vi "Module Loop.vi"(8 "error in (no error)":errorcluster, 11 "Historian Charting Manager in":refnum<class "Historian Charting Manager.lvclass">) -> (0 "error out":errorcluster, 3 "Historian Charting Manager out":refnum<class "Historian Charting Manager.lvclass">)   [LabVIEW 2020, in "VolatusGUI.lvlib" / "Historian Charting Manager.lvclass"]
uses:
  Historian Charting Manager.lvclass
  C:/dev/lv20CE/relink/lv-volatus/Volatus/Module/Module.lvclass
  Volatus/Module/Module.lvclass/Module.ctl
  Volatus/MessageQ/MessageQ.lvclass/MessageQ.ctl
  Charting Config Value/Charting Config Value.lvclass
  Duplicate Group.ctl
  Volatus/Module/Module.lvclass
  Historian Charting Manager.lvclass/Historian Charting Manager.ctl
  JSON Charting Config.ctl
  JSON Chart Group.ctl
  JSON Plot Group.ctl
  JSON Plot Config.ctl
  New Plot Group Data.ctl
  VolatusConfig/VolatusConfigElement/VolatusConfigElement.lvclass
  Chart Info.ctl
  Volatus/MessageQ/MessageQ.lvclass
  Select Plot Group Data.ctl
  Plot Group Config.ctl
  X-Axis Type.ctl
  Plot Config.ctl
  Scale.ctl
  Chart Selection.ctl
  Chart Registration.ctl
  Plot Group Events Value/Plot Group Events Value.lvclass/Plot Group Events Value.ctl
  Plot Group Removed Data.ctl
  VolatusHistorian/Historian Identity/Historian Identity.lvclass
  C:/dev/lv20CE/relink/lv-volatus/Volatus/Identity/Identity.lvclass
  PluginGUI/PluginGUI.lvclass
  Chart GUI.vi
  <vilib>/Utility/error.llb/Error Cluster From Error Code.vi
  lv-promises/Promises/Promise/Promise.lvclass
  Plot Group Events Value/Plot Group Events Value.lvclass
  GUI Helper/GUI Helper.lvclass
  Volatus/Volatus.lvlib
  Volatus/VolatusAPI/VolatusAPI.lvclass
  C:/dev/lv20CE/relink/lv-volatus/VolatusGUI/Historian Charting Manager/Historian Charting Manager.lvclass
  VolatusGUI.lvlib
  GUI Info.ctl
  C:/dev/lv20CE/relink/lv-volatus/VolatusHistorian/Historian Identity/Historian Identity.lvclass
  C:/dev/lv20CE/relink/lv-volatus/VolatusGUI/PluginGUI/PluginGUI.lvclass
panel:
  out "Cover":string
  in  "Export":bool
  in  "Import":bool
  in  "New Chart":bool
  in  "Remove Group":bool
  in  "Dup Group":bool
  in  "New Group":bool
  in  "Chart Group":string(combo)
  # "To configure channels to plot, create a chart and then use the Config button in the upper right of the new chart window to create a plot group."
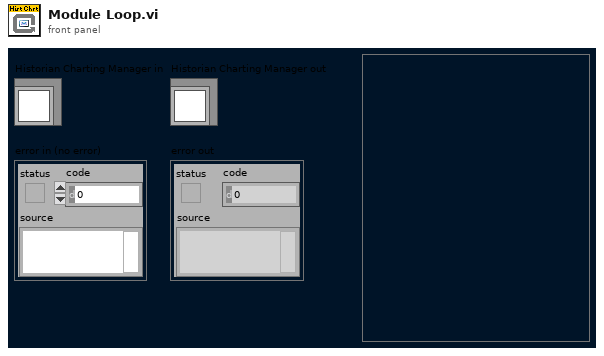
[diagram p1: front panel]
types:
  T1 = typedef "VolatusGUI.lvlib/Historian Charting Manager.lvclass/Duplicate Group.ctl" = cluster{"From":string, "Name":string}
  T2 = typedef "VolatusGUI.lvlib/JSON Charting Config.ctl" = cluster{"ChartGroups":T3[], "PlotGroups":T4[]}
  T3 = typedef "VolatusGUI.lvlib/JSON Chart Group.ctl" = cluster{"Name":string, "PlotGroups":string[]}
  T4 = typedef "VolatusGUI.lvlib/JSON Plot Group.ctl" = cluster{"Name":string, "Chart":cluster{"X-Axis":string, "X-Channel":string, "Now":bool, "Time":string, "SwapAxes":bool}, "Plots":T5[]}
  T5 = typedef "VolatusGUI.lvlib/JSON Plot Config.ctl" = cluster{"Channel":string, "Visible":bool, "Color":string, "Scale":string}
  T6 = enum32{"Invalid", "Standard", "Closed", "Hidden", "Minimized", "Maximized"}
  T7 = typedef "VolatusGUI.lvlib/GUI Info.ctl" = cluster{"Color":u32, "Name":string}
  T8 = enum8{"Enabled", "Disabled", "Disabled and Grayed Out"}
  T9 = typedef "VolatusGUI.lvlib/Historian Charting Manager.lvclass/New Plot Group Data.ctl" = cluster{"Name":string, "Plot Groups":string[]}
  T10 = typedef "VolatusGUI.lvlib/Historian Charting Manager.lvclass/Chart Info.ctl" = cluster{"PluginGUI":refnum<class "MessageQ.lvclass">, "Select Plot Group":refnum<user-event>}
  T11 = typedef "VolatusGUI.lvlib/Historian Charting Manager.lvclass/Select Plot Group Data.ctl" = cluster{"Chart Num":i32, "Plots Config":T12, "Plot Groups":string[]}
  T12 = typedef "VolatusGUI.lvlib/Historian Charting Manager.lvclass/Plot Group Config.ctl" = cluster{"Name":string, "X-Axis Type":T13, "X-Axis Channel":string, "Plots":T14[], "Lock Now":bool, "Time":string, "Swap Axes":bool}
  T13 = typedef "VolatusGUI.lvlib/Historian Charting Manager.lvclass/X-Axis Type.ctl" = enum16{"Time", "Channel"}
  T14 = typedef "VolatusGUI.lvlib/Historian Charting Manager.lvclass/Plot Config.ctl" = cluster{"Channel":string, "Visible":bool, "Color":u32, "Scale":T15}
  T15 = typedef "VolatusGUI.lvlib/Historian Charting Manager.lvclass/Scale.ctl" = enum16{"Left", "Right"}
  T16 = typedef "VolatusGUI.lvlib/Historian Charting Manager.lvclass/Chart Selection.ctl" = cluster{"Chart Num":i32, "Plot Group":string}
  T17 = typedef "VolatusGUI.lvlib/Historian Charting Manager.lvclass/Chart Registration.ctl" = cluster{"Chart Num":i32, "Select Plot Group":refnum<user-event>}
  T18 = typedef "VolatusGUI.lvlib/Historian Charting Manager.lvclass/Plot Group Removed Data.ctl" = cluster{"Name":string, "Plot Groups":string[]}
  T19 = typedef "VolatusGUI.lvlib/Historian Charting Manager.lvclass/Plot Group Events.ctl" = cluster{"Changed":refnum<user-event>, "Removed":refnum<user-event>, "New":refnum<user-event>, "Select":refnum<user-event>}
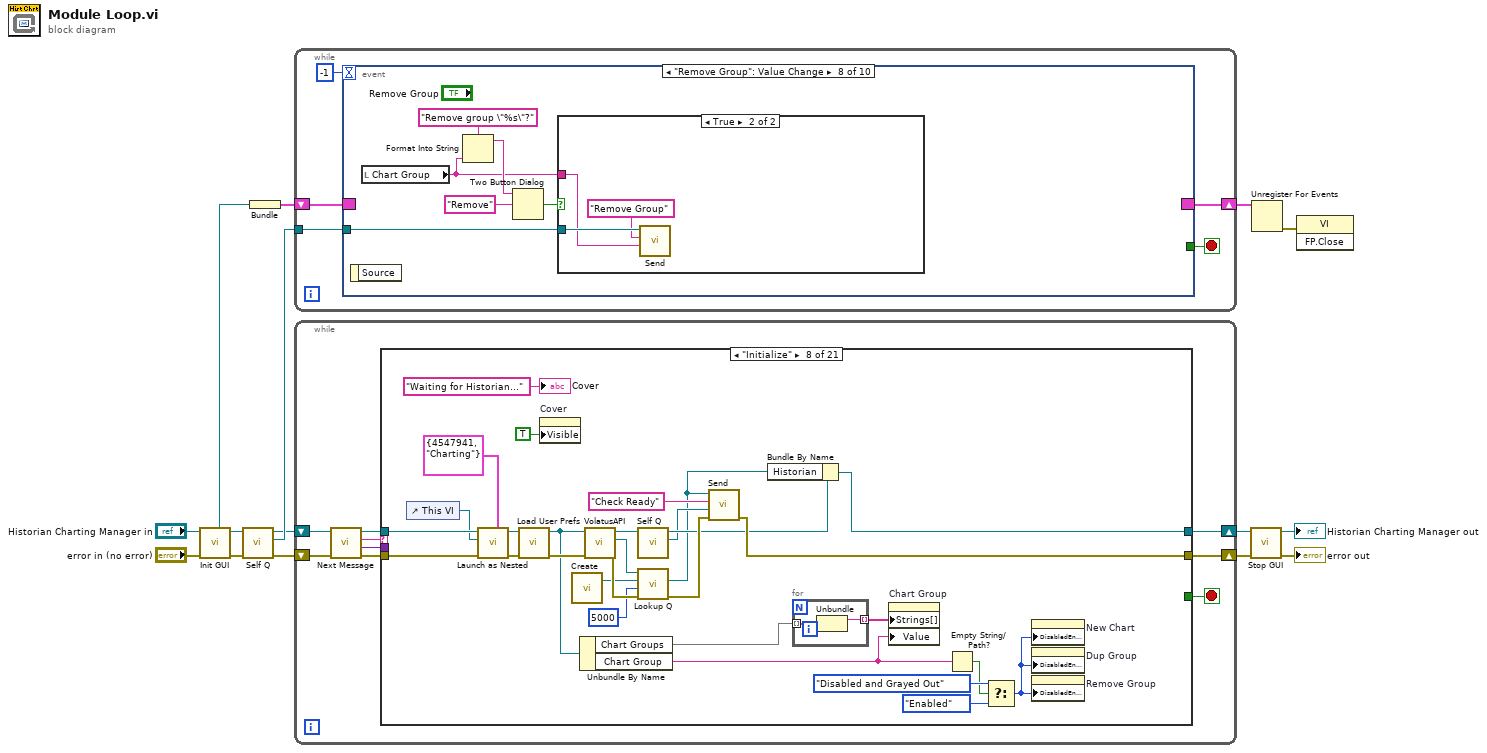
[diagram p0: block diagram]
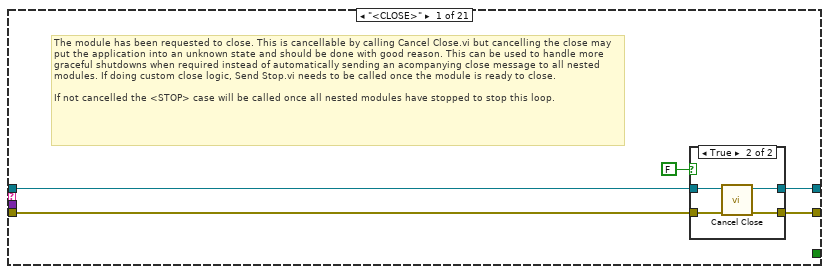
[diagram p2: hidden frame]
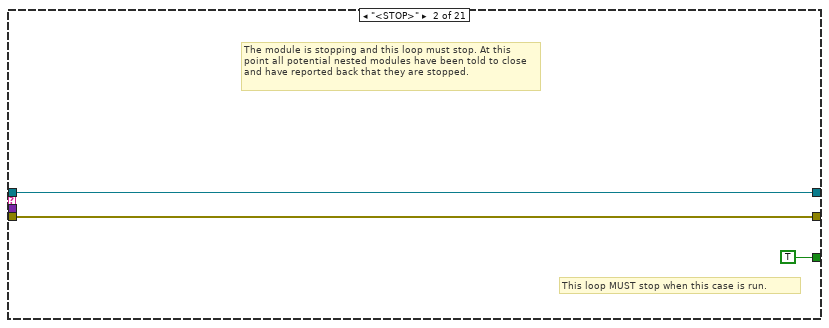
[diagram p4: hidden frame]
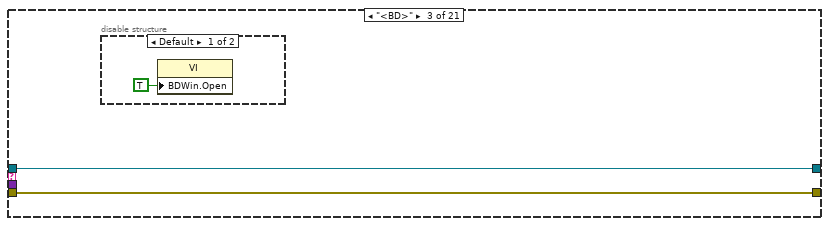
[diagram p5: hidden frame]
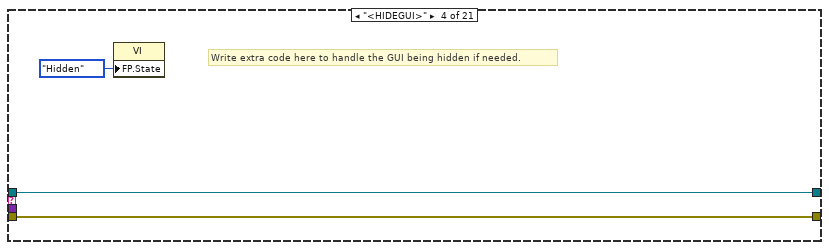
[diagram p7: hidden frame]
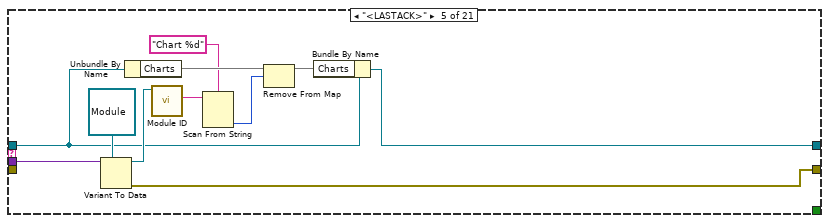
[diagram p8: hidden frame]
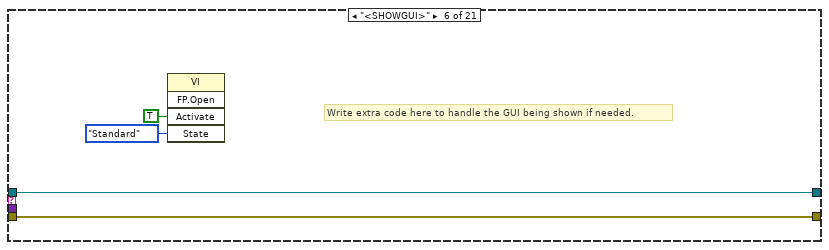
[diagram p9: hidden frame]
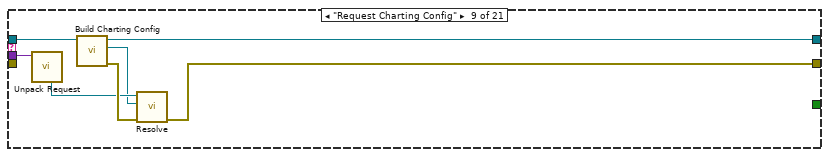
[diagram p11: hidden frame]
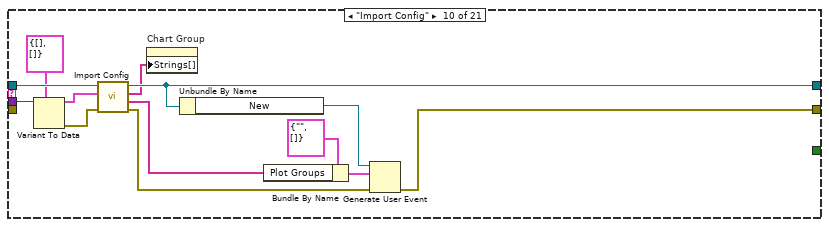
[diagram p12: hidden frame]
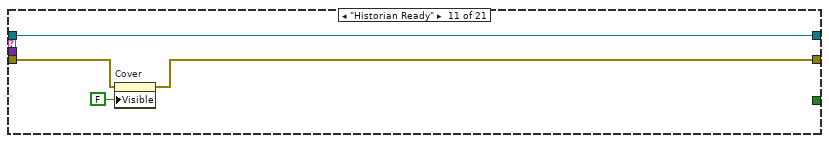
[diagram p13: hidden frame]
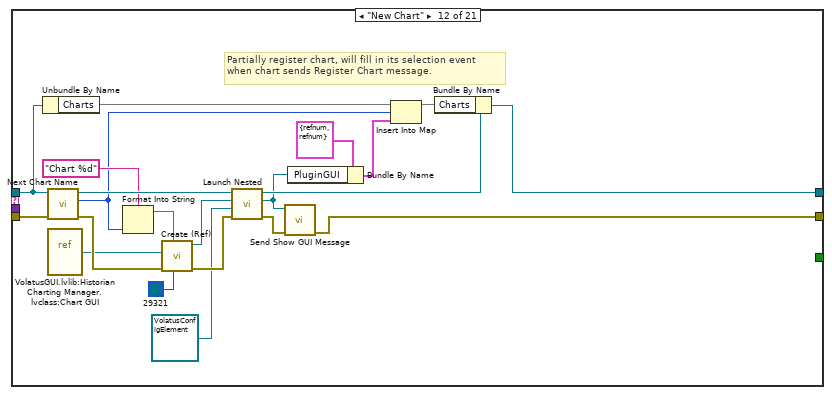
[diagram p14: hidden frame]
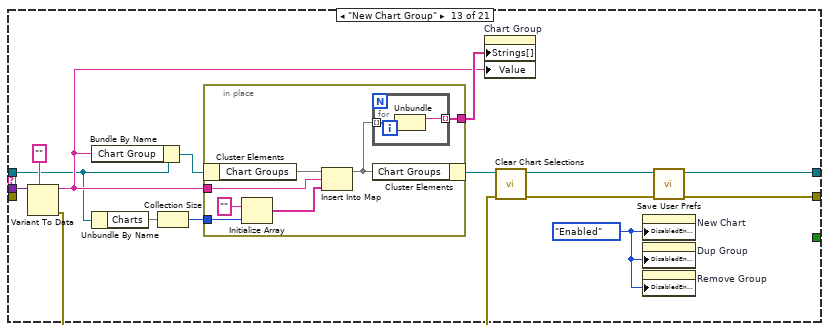
[diagram p15: hidden frame]
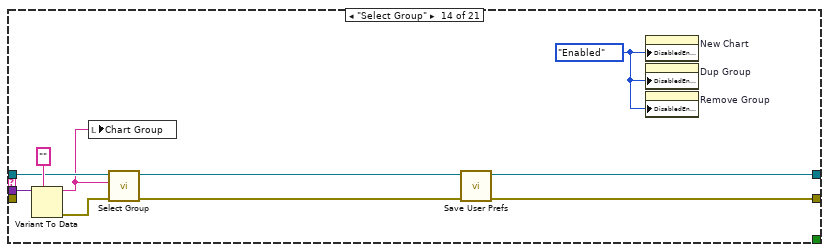
[diagram p16: hidden frame]
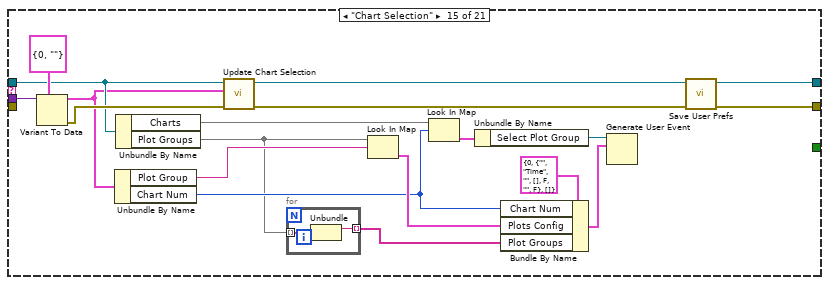
[diagram p17: hidden frame]
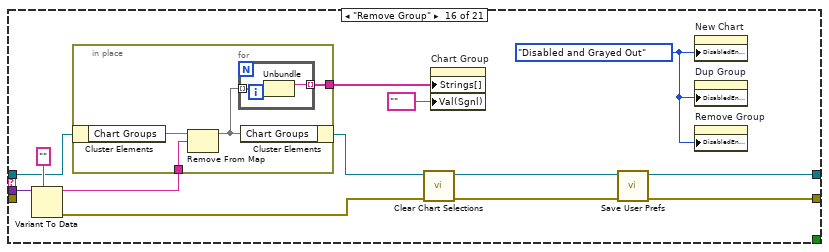
[diagram p18: hidden frame]
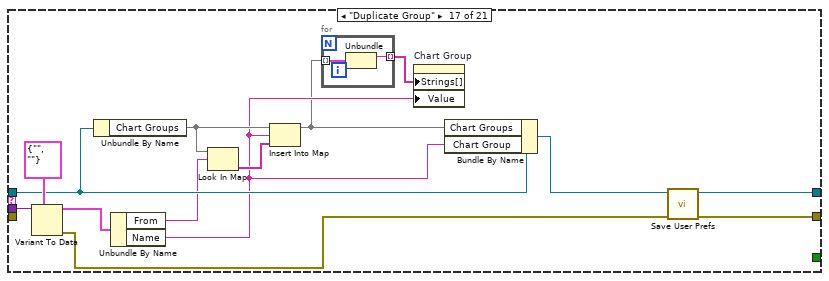
[diagram p19: hidden frame]
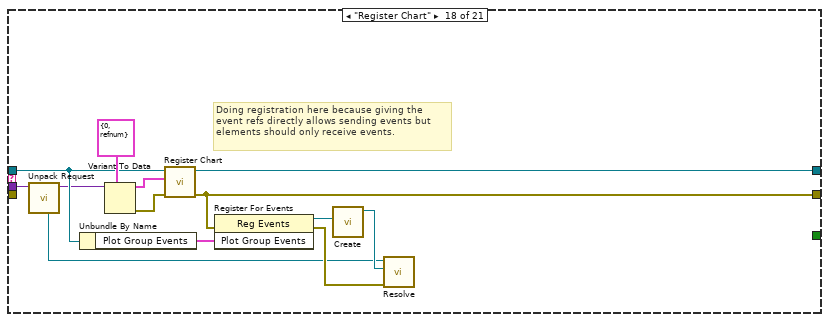
[diagram p20: hidden frame]
diagram:
  n1 = call "Init GUI.vi"("Module in"="Historian Charting Manager in") -> ("Module out"=w7:refnum<class "Historian Charting Manager.lvclass">, "Event Reg"=w12:refnum<event-registration>)  [unwired: 9 in]
  n2 = call "Self Q.vi"("Module in"=w7) -> ("Self Q"=w6:refnum<class "MessageQ.lvclass">, "Module out"=w5:refnum<class "Historian Charting Manager.lvclass">)  [unwired: 9 in]
  n3 = Bundle("Event Reg"=w12) -> (w8:cluster{"Event Reg":refnum<event-registration>})  [unwired: 1 in]
  n4 = while {
    tunnel: w6 -> [w18]
    shift-right: [w16] -> w9
    shift-left: w8 -> [w17]
    stop <- w15 stop-if-true
    n5 = event shown="[7] \"Remove Group\": Value Change" {
      selector: w17 -> [_ _ _ _ _ _ _ _ _ _]
      dyn-events: [_ _ _ _ _ _ _ _ _ _] -> w16
      timeout: -1 -> [_ _ _ _ _ _ _ _ _ _]
      tunnel: w18 -> [_ _ w22 w23 w30 w34 w44 w54 w63 w65]
      tunnel: [_ TRUE _ _ _ _ _ _ _ _] -> w15
      event Timeout {
        n6 = event-data() -> ()  [unwired: 1 in, 1 out]
      }
      event User Event {
        n7 = event-data() -> ()  [unwired: 1 in, 1 out]
      }
      event "Chart Group": Value Change {
        n8 = event-data() -> ("NewVal"=w21:string)  [unwired: 1 in]
        n9 = call "Send.vi"("Data"=w21, "ID"="Select Group", "MessageQ in"=w22) -> ()  [unwired: 7 in, 2 out]
      }
      event "Import": Value Change {
        # "Doing the prompt UI stuff here to allow other messages to still be handled by the QMH loop."
        n10 = event-data() -> ()  [unwired: 1 in, 1 out]
        n11 = call "Import Config UI.vi"() -> ("Config"=w24:T2, "Cancelled"=w25:bool)  [unwired: 10 in]
        n12 = case shown="False" w25 {
          tunnel: w24 -> [w27 _]
          tunnel: w23 -> [w28 _]
          frame False {
            n13 = call "Send.vi"("Data"=w27, "ID"="Import Config", "MessageQ in"=w28) -> ()  [unwired: 7 in, 2 out]
          }
          frame True {
          }
        }
      }
      event "Export": Value Change {
        n14 = event-data() -> ()  [unwired: 1 in, 1 out]
        n15 = call "Request.vi"("Response Type (None)"=refnum<class "Charting Config Value.lvclass"> refnum ("VolatusGUI:Charting Config Value.lvclass"), "ID"="Request Charting Config", "MessageQ in"=w30) -> ("Response"=w31:refnum<class "Charting Config Value.lvclass">)  [unwired: 6 in, 2 out]
        n16 = call "Read.vi"("Charting Config Value in"=w31) -> ("JSON Charting Config"=w29:T2)  [unwired: 10 in]
        n17 = call "Export Config UI.vi"("Config"=w29) -> ()  [unwired: 11 in]
      }
      event "New Group": Value Change {
        n18 = event-data() -> ()  [unwired: 1 in, 1 out]
        n19 = call "Group Name Prompt.vi"("Prompt"="Enter name for new group:") -> ("Cancelled"=w36:bool, "Name"=w35:string)  [unwired: 9 in]
        n20 = case shown="False" w36 {
          tunnel: w35 -> [w38 _]
          tunnel: w34 -> [w40 _]
          frame False {
            n21 = call "Send.vi"("Data"=w38, "ID"="New Chart Group", "MessageQ in"=w40) -> ()  [unwired: 7 in, 2 out]
          }
          frame True {
          }
        }
      }
      event "Dup Group": Value Change {
        n22 = event-data() -> ()  [unwired: 1 in, 1 out]
        n23 = local read "Chart Group"() -> (w42:string)
        n24 = Format Into String(format string="Enter new name for duplicated \"%s\" group:", w42) -> (resulting string=w41:string)  [unwired: 2 in, 1 out]
        n25 = call "Group Name Prompt.vi"("Prompt"=w41) -> ("Cancelled"=w45:bool, "Name"=w46:string)  [unwired: 9 in]
        n26 = case shown="False" w45 {
          tunnel: w46 -> [w50 _]
          tunnel: w44 -> [w49 _]
          tunnel: w42 -> [w51 _]
          frame False {
            n27 = Bundle By Name(cluster=T1 {"From"="", "Name"=""} ("Duplicate Group"), "From"=w51, "Name"=w50) -> (w48:T1)
            n28 = call "Send.vi"("Data"=w48, "ID"="Duplicate Group", "MessageQ in"=w49) -> ()  [unwired: 7 in, 2 out]
          }
          frame True {
          }
        }
      }
      event "Remove Group": Value Change {
        n29 = event-data() -> ()  [unwired: 1 in, 1 out]
        n30 = local read "Chart Group"() -> (w53:string)
        n31 = Format Into String(format string="Remove group \"%s\"?", w53) -> (resulting string=w56:string)  [unwired: 2 in, 1 out]
        n32 = Two Button Dialog(message=w56, 2:"Remove" ("T button name (\"OK\")")) -> (T button?=w55:bool)  [unwired: 1 in]
        n33 = case shown="True" w55 {
          tunnel: w54 -> [_ w61]
          tunnel: w53 -> [_ w59]
          frame False {
          }
          frame True {
            n34 = call "Send.vi"("Data"=w59, "ID"="Remove Group", "MessageQ in"=w61) -> ()  [unwired: 7 in, 2 out]
          }
        }
      }
      event "New Chart": Value Change {
        n35 = event-data() -> ()  [unwired: 1 in, 1 out]
        n36 = call "Send.vi"("ID"="New Chart", "MessageQ in"=w63) -> ()  [unwired: 8 in, 2 out]
      }
      event Panel Close? {
        n37 = event-data() -> ()  [unwired: 1 in, 1 out]
        n38 = call "Send.vi"("ID"="<HIDEGUI>", "MessageQ in"=w65) -> ()  [unwired: 8 in, 2 out]
        n39 = event-data("Discard?"=TRUE) -> ()  [unwired: 1 in, 1 out]
      }
    }
  }
  n40 = while {
    shift-right: [w70] -> w10
    shift-left: w5 -> [w75]
    shift-right: [w67] -> w11
    shift-left: "error in (no error)" -> [w74]
    stop <- w69 stop-if-true
    n41 = call "Next Message.vi"("error in (no error)"=w74, "Module in"=w75) -> ("error out"=w73:errorcluster, "Data"=w68:variant, "ID"=w72:string, "Module out"=w71:refnum<class "Historian Charting Manager.lvclass">)  [unwired: 6 in]
    n42 = case shown="\"Initialize\"" w72 {
      tunnel: w73 -> [w78 w88 w90 w94 _ w109 w111 w137 _ _ w164 w185 _ _ _ _ _ _ _ _ w321]
      tunnel: w71 -> [w79 w89 w91 w95 w101 w110 w112 w135 w147 w162 w166 w174 w190 w216 w225 w252 w273 w281 w299 w309 w319]
      tunnel: [w77 w89 w91 w95 w99 w110 w112 w117 w146 w157 w166 w171 w193 w212 w227 w244 w264 w286 w291 w301 w318] -> w70
      tunnel: [_ TRUE _ _ _ _ _ _ _ _ _ _ _ _ _ _ _ _ _ _ _] -> w69
      tunnel: w68 -> [_ _ _ _ w106 _ _ _ w148 w161 _ _ w202 w221 w239 w255 w275 w282 w298 w311 _]
      tunnel: [w76 w88 w90 w94 w104 w109 w111 w138 w143 w150 w163 w178 w195 w214 w226 w246 w262 w278 w293 w302 w320] -> w67
      frame "<CLOSE>" {
        # "The module has been requested to close. This is cancellable by calling Cancel Close.vi but cancelling the close may put the application into an unknown state and should be done with good reason. This can be used to handle more graceful shutdowns when required instead of automatically sending an acompanying close message to all nested modules. If doing custom close logic, Send Stop.vi needs to be called once the module is ready to close.\n\nIf not cancelled the <STOP> case will be called once all nested modules have stopped to stop this loop."
        n43 = case shown="True" FALSE {
          tunnel: w78 -> [w81 w86]
          tunnel: [w81 w85] -> w76
          tunnel: w79 -> [w82 w84]
          tunnel: [w82 w83] -> w77
          frame False {
          }
          frame True {
            n44 = call "Cancel Close.vi"("error in (no error)"=w86, "Module in"=w84) -> ("error out"=w85:errorcluster, "Module out"=w83:refnum<class "Historian Charting Manager.lvclass">)  [unwired: 8 in]
          }
        }
      }
      frame "<STOP>" {
        # "This loop MUST stop when this case is run."
        # "The module is stopping and this loop must stop. At this point all potential nested modules have been told to close and have reported back that they are stopped."
      }
      frame "<BD>" {
        n45 = disable-structure shown="Default" {
          frame condition #0 (active) {
            n46 = property class="VI"("BDWin.Open"=TRUE ("Block Diagram Window:Open")) -> ()  [unwired: 2 in, 2 out]
          }
          frame condition #1 {
          }
        }
      }
      frame "<HIDEGUI>" {
        # "Write extra code here to handle the GUI being hidden if needed."
        n47 = property class="VI"("FP.State"=T6."Hidden" ("Front Panel Window:State")) -> ()  [unwired: 2 in, 2 out]
      }
      frame "<LASTACK>" {
        n48 = Variant To Data(type=refnum<class "Module.lvclass"> refnum ("Volatus:Module"), Variant=w106) -> (data=w103:refnum<class "Module.lvclass">, error out=w104:errorcluster)  [unwired: 1 in]
        n49 = Unbundle By Name(w101) -> ("Charts"=w102:map{i32, T10})
        n50 = call-dynamic "Module ID.vi"("Module in"=w103) -> ("Module ID"=w98:string)  [unwired: 10 in]
        n51 = Scan From String(format string="Chart %d", input string=w98) -> (output 1=w96:i32)  [unwired: 3 in, 3 out]
        n52 = Remove From Map(10:w96, 11:w102) -> (3:w100:map{i32, T10})  [unwired: 2 out]
        n53 = Bundle By Name(cluster=w101, "Charts"=w100) -> (w99:refnum<class "Historian Charting Manager.lvclass">)
      }
      frame "<SHOWGUI>" {
        # "Write extra code here to handle the GUI being shown if needed."
        n54 = invoke class="VI" method="FP.Open"("Activate"=TRUE ("Activate?"), "State"=T6."Standard") -> ()  [unwired: 3 in, 5 out]
      }
      frame "<TIMEOUT>" {
        # "No message for this module was received in time"
      }
      frame "Initialize" {
        n55 = control-ref of="This VI"() -> (w134:refnum<vi>)
        n56 = call "Launch as Nested.vi"("GUI Info (Default)"=T7 {"Color"=4547941, "Name"="Charting"}, "error in (no error)"=w137, "GUI"=w134, "Parent in"=w135) -> ("error out"=w136:errorcluster, "Parent"=w133:refnum<class "Historian Charting Manager.lvclass">)  [unwired: 5 in, 1 out]
        n57 = call "Load User Prefs.vi"("error in (no error)"=w136, "Historian Charting Manager in"=w133) -> ("error out"=w139:errorcluster, "Historian Charting Manager out"=w126:refnum<class "Historian Charting Manager.lvclass">)  [unwired: 8 in]
        n58 = property on="Cover" class="Str"("Visible"=TRUE) -> ()  [unwired: 2 in, 2 out]
        n59 = call "Create.vi"() -> ("Historian Identity out"=w120:refnum<class "Historian Identity.lvclass">)  [unwired: 7 in]
        n60 = Unbundle By Name(w126) -> ("Chart Groups"=w132:map{string, string[]}, "Chart Group"=w128:string)
        n61 = call "VolatusAPI.vi"("Module in"=w126) -> ("VolatusAPI"=w118:refnum<class "VolatusAPI.lvclass">, "Module out"=w119:refnum<class "Historian Charting Manager.lvclass">)  [unwired: 9 in]
        n62 = call "Self Q.vi"("Module in"=w119) -> ("Self Q"=w124:refnum<class "MessageQ.lvclass">, "Module out"=w125:refnum<class "Historian Charting Manager.lvclass">)  [unwired: 9 in]
        n63 = call "Lookup Q.vi"("error in (no error)"=w139, "Timeout ms (0)"=5000, "Identity"=w120, "VolatusAPI in"=w118) -> ("error out"=w140:errorcluster, "MessageQ"=w116:refnum<class "MessageQ.lvclass">)  [unwired: 5 in, 1 out]
        n64 = call "Send.vi"("error in (no error)"=w140, "Data"=w124, "ID"="Check Ready", "MessageQ in"=w116) -> ("error out"=w138:errorcluster)  [unwired: 6 in, 1 out]
        n65 = Bundle By Name(cluster=w125, "Historian"=w116) -> (w117:refnum<class "Historian Charting Manager.lvclass">)
        n66 = for {
          tunnel: w132 -> [w142] mode=indexing
          tunnel: [w141] -> w131 mode=indexing
          n67 = Unbundle(w142) -> ("Chart Group"=w141:string)  [unwired: 1 out]
        }
        n68 = property on="Chart Group" class="CmbBox"("Strings[]"=w131, "Value"=w128) -> ()  [unwired: 2 in, 2 out]
        n69 = Empty String/Path?(string/path=w128) -> (empty?=w127:bool)
        n70 = Select(t=T8."Disabled and Grayed Out" ("Disabled"), s=w127, f=T8."Enabled") -> (s? t:f=w114:T8)
        n71 = property on="New Chart" class="Bool"("DisabledEnum"=w114) -> ()  [unwired: 2 in, 2 out]
        n72 = property on="Dup Group" class="Bool"("DisabledEnum"=w114) -> ()  [unwired: 2 in, 2 out]
        n73 = property on="Remove Group" class="Bool"("DisabledEnum"=w114) -> ()  [unwired: 2 in, 2 out]
        "Cover" <- "Waiting for Historian..." ("Cover")
      }
      frame "Request Charting Config" {
        n74 = call "Unpack Request.vi"("Request Data"=w148) -> ("Promise"=w145:refnum<class "Promise.lvclass">)  [unwired: 8 in, 2 out]
        n75 = call "Build Charting Config.vi"("Historian Charting Manager in"=w147) -> ("error out"=w149:errorcluster, "Charting Config Value"=w144:refnum<class "Charting Config Value.lvclass">, "Historian Charting Manager out"=w146:refnum<class "Historian Charting Manager.lvclass">)  [unwired: 8 in]
        n76 = call "Resolve.vi"("error in (no error)"=w149, "Result (None)"=w144, "Promise in"=w145) -> ("error out"=w143:errorcluster)  [unwired: 7 in, 1 out]
      }
      frame "Import Config" {
        n77 = Variant To Data(type=T2 {"ChartGroups"=[], "PlotGroups"=[]} ("JSON Charting Config"), Variant=w161) -> (data=w159:T2, error out=w158:errorcluster)  [unwired: 1 in]
        n78 = call "Import Config.vi"("error in (no error)"=w158, "JSON Charting Config"=w159, "Historian Charting Manager in"=w162) -> ("error out"=w151:errorcluster, "Plot Groups"=w153:string[], "Chart Groups"=w152:string[], "Historian Charting Manager out"=w157:refnum<class "Historian Charting Manager.lvclass">)  [unwired: 5 in]
        n79 = property on="Chart Group" class="CmbBox"("Strings[]"=w152) -> ()  [unwired: 2 in, 2 out]
        n80 = Unbundle By Name(w157) -> ("New"=w156:refnum<user-event>)
        n81 = Bundle By Name(cluster=T9 {"Name"="", "Plot Groups"=[]} ("event data"), "Plot Groups"=w153) -> (w154:T9)
        n82 = Generate User Event(user event=w156, event data cluster=w154, error in=w151) -> (error out=w150:errorcluster)  [unwired: 1 in, 1 out]
      }
      frame "Historian Ready" {
        n83 = property on="Cover" class="Str"(error in=w164, "Visible"=FALSE) -> (error out=w163:errorcluster)  [unwired: 1 in, 1 out]
      }
      frame "New Chart" {
        # "Partially register chart, will fill in its selection event when chart sends Register Chart message."
        n84 = Unbundle By Name(w174) -> ("Charts"=w173:map{i32, T10})
        n85 = call "Next Chart Name.vi"("error in (no error)"=w185, "Historian Charting Manager in"=w174) -> ("error out"=w186:errorcluster, "Next Chart Num"=w169:i32, "Historian Charting Manager out"=w183:refnum<class "Historian Charting Manager.lvclass">)  [unwired: 7 in]
        n86 = vi-ref "VolatusGUI.lvlib:Historian Charting Manager.lvclass:Chart GUI.vi"() -> (w184:refnum<vi>)
        n87 = Format Into String(format string="Chart %d", w169) -> (resulting string=w175:string)  [unwired: 2 in, 1 out]
        n88 = call "Create (Ref).vi"("Color (Default)"=u32 29321, "Name"=w175, "error in (no error)"=w186, "VI"=w184) -> ("error out"=w187:errorcluster, "PluginGUI out"=w182:refnum<class "PluginGUI.lvclass">)  [unwired: 6 in]
        n89 = call "Launch Nested.vi"("error in (no error)"=w187, "Config Element"=refnum<class "VolatusConfigElement.lvclass"> refnum, "Nested Module"=w182, "Parent in"=w183) -> ("error out"=w179:errorcluster, "MessageQ"=w167:refnum<class "MessageQ.lvclass">, "Parent out"=w180:refnum<class "Historian Charting Manager.lvclass">)  [unwired: 5 in]
        n90 = call "Send Show GUI Message.vi"("error in (no error)"=w179, "MessageQ"=w167) -> ("error out"=w178:errorcluster)  [unwired: 9 in]
        n91 = Bundle By Name(cluster=T10 {"PluginGUI"=refnum, "Select Plot Group"=refnum} ("value"), "PluginGUI"=w167) -> (w168:T10)
        n92 = Insert Into Map(map in=w173, key=w169, value=w168) -> (map out=w170:map{i32, T10})  [unwired: 2 out]
        n93 = Bundle By Name(cluster=w180, "Charts"=w170) -> (w171:refnum<class "Historian Charting Manager.lvclass">)
      }
      frame "New Chart Group" {
        w192 = T8."Enabled" ("Disabled")
        n94 = Variant To Data(type="", Variant=w202) -> (data=w191:string, error out=w200:errorcluster)  [unwired: 1 in]
        n95 = Bundle By Name(cluster=w190, "Chart Group"=w191) -> (w196:refnum<class "Historian Charting Manager.lvclass">)
        n96 = Unbundle By Name(w190) -> ("Charts"=w189:map{i32, T10})
        n97 = Collection Size(1:w189) -> (0:w188:i32)
        n98 = in-place {
          in-place-border: w191 -> [w208]
          in-place-border: [w206] -> w197
          in-place-border: w188 -> [w205]
          n99 = in-place-cluster #1(w196) -> ("Chart Groups"=w209:map{string, string[]})
          n100 = Initialize Array("", w205) -> (w203:string[])
          n101 = Insert Into Map(map in=w209, key=w208, value=w203) -> (map out=w207:map{string, string[]})  [unwired: 2 out]
          n102 = for {
            tunnel: w207 -> [w211] mode=indexing
            tunnel: [w210] -> w206 mode=indexing
            n103 = Unbundle(w211) -> ("Chart Group"=w210:string)  [unwired: 1 out]
          }
          n104 = in-place-cluster #1("Chart Groups"=w207) -> (w198:refnum<class "Historian Charting Manager.lvclass">)
        }
        n105 = property on="Chart Group" class="CmbBox"("Strings[]"=w197, "Value"=w191) -> ()  [unwired: 2 in, 2 out]
        n106 = call "Clear Chart Selections.vi"("error in (no error)"=w200, "Historian Charting Manager in"=w198) -> ("error out"=w199:errorcluster, "Historian Charting Manager out"=w194:refnum<class "Historian Charting Manager.lvclass">)  [unwired: 8 in]
        n107 = property on="New Chart" class="Bool"("DisabledEnum"=w192) -> ()  [unwired: 2 in, 2 out]
        n108 = property on="Dup Group" class="Bool"("DisabledEnum"=w192) -> ()  [unwired: 2 in, 2 out]
        n109 = property on="Remove Group" class="Bool"("DisabledEnum"=w192) -> ()  [unwired: 2 in, 2 out]
        n110 = call "Save User Prefs.vi"("error in (no error)"=w199, "Historian Charting Manager in"=w194) -> ("error out"=w195:errorcluster, "Historian Charting Manager out"=w193:refnum<class "Historian Charting Manager.lvclass">)  [unwired: 8 in]
      }
      frame "Select Group" {
        w219 = T8."Enabled" ("Disabled")
        n111 = Variant To Data(type="", Variant=w221) -> (data=w215:string, error out=w218:errorcluster)  [unwired: 1 in]
        n112 = local write "Chart Group"(w215) -> ()
        n113 = call "Select Group.vi"("error in (no error)"=w218, "Group (Empty = none)"=w215, "Historian Charting Manager in"=w216) -> ("error out"=w217:errorcluster, "Historian Charting Manager out"=w213:refnum<class "Historian Charting Manager.lvclass">)  [unwired: 7 in]
        n114 = call "Save User Prefs.vi"("error in (no error)"=w217, "Historian Charting Manager in"=w213) -> ("error out"=w214:errorcluster, "Historian Charting Manager out"=w212:refnum<class "Historian Charting Manager.lvclass">)  [unwired: 8 in]
        n115 = property on="New Chart" class="Bool"("DisabledEnum"=w219) -> ()  [unwired: 2 in, 2 out]
        n116 = property on="Dup Group" class="Bool"("DisabledEnum"=w219) -> ()  [unwired: 2 in, 2 out]
        n117 = property on="Remove Group" class="Bool"("DisabledEnum"=w219) -> ()  [unwired: 2 in, 2 out]
      }
      frame "Chart Selection" {
        n118 = Variant To Data(type=T16 {"Chart Num"=0, "Plot Group"=""} ("Chart Selection"), Variant=w239) -> (data=w222:T16, error out=w240:errorcluster)  [unwired: 1 in]
        n119 = Unbundle By Name(w222) -> ("Plot Group"=w231:string, "Chart Num"=w230:i32)
        n120 = Unbundle By Name(w225) -> ("Charts"=w237:map{i32, T10}, "Plot Groups"=w229:map{string, T12})
        n121 = call "Update Chart Selection.vi"("error in (no error)"=w240, "Chart Selection"=w222, "Historian Charting Manager in"=w225) -> ("error out"=w224:errorcluster, "Historian Charting Manager out"=w223:refnum<class "Historian Charting Manager.lvclass">)  [unwired: 7 in]
        n122 = for {
          tunnel: w229 -> [w242] mode=indexing
          tunnel: [w241] -> w228 mode=indexing
          n123 = Unbundle(w242) -> ("Name"=w241:string)  [unwired: 1 out]
        }
        n124 = Look In Map(map=w229, key=w231) -> (value=w232:T12)  [unwired: 1 in, 1 out]
        n125 = Look In Map(map=w237, key=w230) -> (value=w236:T10)  [unwired: 1 in, 1 out]
        n126 = Unbundle By Name(w236) -> ("Select Plot Group"=w235:refnum<user-event>)
        n127 = Bundle By Name(cluster=T11 {"Chart Num"=0, "Plots Config"={"Name"="", "X-Axis Type"=enum."Time", "X-Axis Channel"="", "Plots"=[], "Lock Now"=FALSE, "Time"="", "Swap Axes"=FALSE}, "Plot Groups"=[]} ("event data"), "Chart Num"=w230, "Plots Config"=w232, "Plot Groups"=w228) -> (w233:T11)
        n128 = Generate User Event(user event=w235, event data cluster=w233) -> ()  [unwired: 2 in, 2 out]
        n129 = call "Save User Prefs.vi"("error in (no error)"=w224, "Historian Charting Manager in"=w223) -> ("error out"=w226:errorcluster, "Historian Charting Manager out"=w227:refnum<class "Historian Charting Manager.lvclass">)  [unwired: 8 in]
      }
      frame "Remove Group" {
        w253 = T8."Disabled and Grayed Out" ("Disabled")
        n130 = Variant To Data(type="", Variant=w255) -> (data=w251:string, error out=w249:errorcluster)  [unwired: 1 in]
        n131 = in-place {
          in-place-border: w251 -> [w258]
          in-place-border: [w256] -> w243
          n132 = in-place-cluster #2(w252) -> ("Chart Groups"=w259:map{string, string[]})
          n133 = Remove From Map(10:w258, 11:w259) -> (3:w257:map{string, string[]})  [unwired: 2 out]
          n134 = for {
            tunnel: w257 -> [w261] mode=indexing
            tunnel: [w260] -> w256 mode=indexing
            n135 = Unbundle(w261) -> ("Chart Group"=w260:string)  [unwired: 1 out]
          }
          n136 = in-place-cluster #2("Chart Groups"=w257) -> (w250:refnum<class "Historian Charting Manager.lvclass">)
        }
        n137 = call "Clear Chart Selections.vi"("error in (no error)"=w249, "Historian Charting Manager in"=w250) -> ("error out"=w248:errorcluster, "Historian Charting Manager out"=w245:refnum<class "Historian Charting Manager.lvclass">)  [unwired: 8 in]
        n138 = property on="Chart Group" class="CmbBox"("Strings[]"=w243, "Val(Sgnl)"="" ("Chart Group")) -> ()  [unwired: 2 in, 2 out]
        n139 = call "Save User Prefs.vi"("error in (no error)"=w248, "Historian Charting Manager in"=w245) -> ("error out"=w246:errorcluster, "Historian Charting Manager out"=w244:refnum<class "Historian Charting Manager.lvclass">)  [unwired: 8 in]
        n140 = property on="New Chart" class="Bool"("DisabledEnum"=w253) -> ()  [unwired: 2 in, 2 out]
        n141 = property on="Dup Group" class="Bool"("DisabledEnum"=w253) -> ()  [unwired: 2 in, 2 out]
        n142 = property on="Remove Group" class="Bool"("DisabledEnum"=w253) -> ()  [unwired: 2 in, 2 out]
      }
      frame "Duplicate Group" {
        n143 = Variant To Data(type=T1 {"From"="", "Name"=""} ("Duplicate Group"), Variant=w275) -> (data=w272:T1, error out=w263:errorcluster)  [unwired: 1 in]
        n144 = Unbundle By Name(w273) -> ("Chart Groups"=w270:map{string, string[]})
        n145 = Unbundle By Name(w272) -> ("From"=w271:string, "Name"=w267:string)
        n146 = Look In Map(map=w270, key=w271) -> (value=w269:string[])  [unwired: 1 in, 1 out]
        n147 = Insert Into Map(map in=w270, key=w267, value=w269) -> (map out=w266:map{string, string[]})  [unwired: 2 out]
        n148 = for {
          tunnel: w266 -> [w277] mode=indexing
          tunnel: [w276] -> w265 mode=indexing
          n149 = Unbundle(w277) -> ("Chart Group"=w276:string)  [unwired: 1 out]
        }
        n150 = property on="Chart Group" class="CmbBox"("Strings[]"=w265, "Value"=w267) -> ()  [unwired: 2 in, 2 out]
        n151 = Bundle By Name(cluster=w273, "Chart Groups"=w266, "Chart Group"=w267) -> (w268:refnum<class "Historian Charting Manager.lvclass">)
        n152 = call "Save User Prefs.vi"("error in (no error)"=w263, "Historian Charting Manager in"=w268) -> ("error out"=w262:errorcluster, "Historian Charting Manager out"=w264:refnum<class "Historian Charting Manager.lvclass">)  [unwired: 8 in]
      }
      frame "Register Chart" {
        # "Doing registration here because giving the event refs directly allows sending events but elements should only receive events."
        n153 = call "Unpack Request.vi"("Request Data"=w282) -> ("Data"=w280:variant, "Promise"=w279:refnum<class "Promise.lvclass">)  [unwired: 8 in, 1 out]
        n154 = Unbundle By Name(w281) -> ("Plot Group Events"=w284:T19)
        n155 = Variant To Data(type=T17 {"Chart Num"=0, "Select Plot Group"=refnum} ("Chart Registration"), Variant=w280) -> (data=w288:T17, error out=w287:errorcluster)  [unwired: 1 in]
        n156 = call "Register Chart.vi"("error in (no error)"=w287, "Chart Registration"=w288, "Historian Charting Manager in"=w281) -> ("error out"=w278:errorcluster, "Historian Charting Manager out"=w286:refnum<class "Historian Charting Manager.lvclass">)  [unwired: 7 in]
        n157 = register-events(error in=w278, w284) -> (reference out=w283:refnum<event-registration>, error out=w290:errorcluster)  [unwired: 1 in]
        n158 = call "Create.vi"("Plot Group"=w283) -> ("Plot Group Events Value out"=w285:refnum<class "Plot Group Events Value.lvclass">)  [unwired: 10 in]
        n159 = call "Resolve.vi"("error in (no error)"=w290, "Result (None)"=w285, "Promise in"=w279) -> ()  [unwired: 7 in, 2 out]
      }
      frame "Update Plots Config" {
        n160 = Variant To Data(type=T12 {"Name"="", "X-Axis Type"=enum."Time", "X-Axis Channel"="", "Plots"=[], "Lock Now"=FALSE, "Time"="", "Swap Axes"=FALSE} ("Plot Group Config"), Variant=w298) -> (data=w296:T12, error out=w295:errorcluster)  [unwired: 1 in]
        n161 = call "Update Plots Config.vi"("error in (no error)"=w295, "Plot Group Config"=w296, "Historian Charting Manager in"=w299) -> ("error out"=w294:errorcluster, "Historian Charting Manager out"=w292:refnum<class "Historian Charting Manager.lvclass">)  [unwired: 7 in]
        n162 = call "Save User Prefs.vi"("error in (no error)"=w294, "Historian Charting Manager in"=w292) -> ("error out"=w293:errorcluster, "Historian Charting Manager out"=w291:refnum<class "Historian Charting Manager.lvclass">)  [unwired: 8 in]
      }
      frame "Remove Plot Group" {
        n163 = Variant To Data(type="", Variant=w311) -> (data=w303:string)  [unwired: 1 in, 1 out]
        n164 = in-place {
          in-place-border: w303 -> [w314]
          in-place-border: [w312] -> w304
          n165 = in-place-cluster #3(w309) -> ("Plot Groups"=w315:map{string, T12})
          n166 = Remove From Map(10:w314, 11:w315) -> (3:w313:map{string, T12})  [unwired: 2 out]
          n167 = in-place-cluster #3("Plot Groups"=w313) -> (w300:refnum<class "Historian Charting Manager.lvclass">)
          n168 = for {
            tunnel: w313 -> [w317] mode=indexing
            tunnel: [w316] -> w312 mode=indexing
            n169 = Unbundle(w317) -> ("Name"=w316:string)  [unwired: 1 out]
          }
        }
        n170 = Bundle By Name(cluster=T18 {"Name"="", "Plot Groups"=[]} ("event data"), "Plot Groups"=w304, "Name"=w303) -> (w306:T18)
        n171 = Unbundle By Name(w300) -> ("Removed"=w308:refnum<user-event>)
        n172 = Generate User Event(user event=w308, event data cluster=w306) -> (error out=w305:errorcluster)  [unwired: 2 in, 1 out]
        n173 = call "Save User Prefs.vi"("error in (no error)"=w305, "Historian Charting Manager in"=w300) -> ("error out"=w302:errorcluster, "Historian Charting Manager out"=w301:refnum<class "Historian Charting Manager.lvclass">)  [unwired: 8 in]
      }
      frame Default {
        n174 = call "Report Unhandled Message ID.vi"("error in (no error)"=w321, "Module in"=w319) -> ("error out"=w320:errorcluster, "Module out"=w318:refnum<class "Historian Charting Manager.lvclass">)  [unwired: 8 in]
      }
    }
  }
  n175 = call "Stop GUI.vi"("error in (no error)"=w11, "Module in"=w10) -> ("error out"=→"error out":errorcluster, "Module out"=→"Historian Charting Manager out":refnum<class "Historian Charting Manager.lvclass">)  [unwired: 8 in]
  n176 = Unregister For Events(event registration refnum=w9) -> (error out=w13:errorcluster)  [unwired: 1 in]
  n177 = invoke class="VI" method="FP.Close"(error in=w13) -> ()  [unwired: 2 in, 3 out]
